vi "Create Paragraph Collection.vi"(8 "error in (no error)":errorcluster, 10 "Text":string, 11 "ooWriter in":refnum<class "ooWriter.lvclass">) -> (0 "error out":errorcluster, 2 "Paragraph Collection":refnum<k24>, 3 "ooWriter out":refnum<class "ooWriter.lvclass">)   [LabVIEW 2009, in "ooWriter.lvclass"]
uses:
  ooWriter.lvclass
  C:/Projets/LAVAG/OpenOfficeRGT/AODL/DLLs/AODL.dll
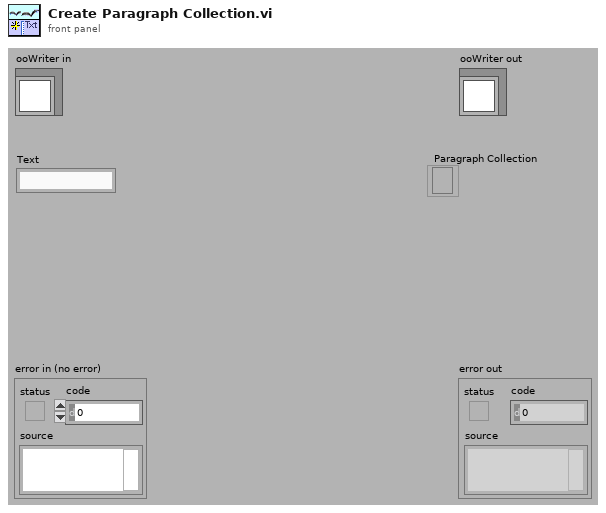
[diagram p1: front panel]
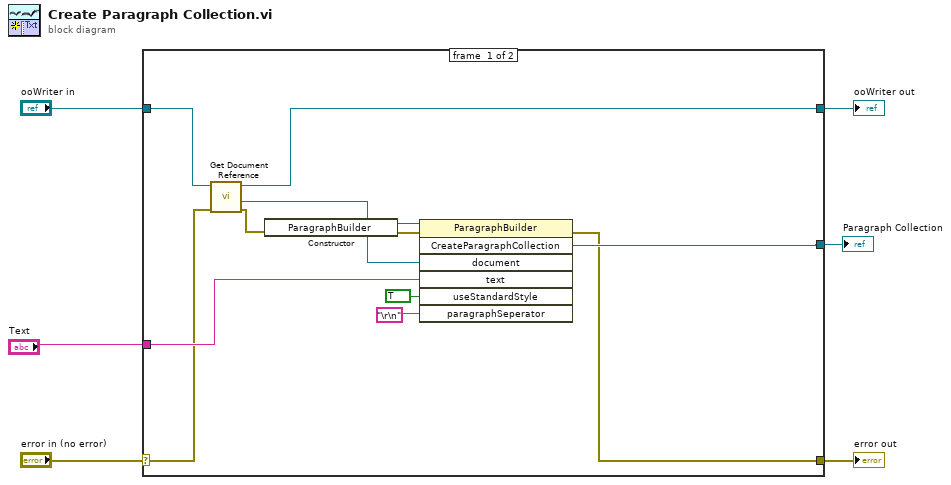
[diagram p0: block diagram]
diagram:
  n1 = case shown="No Error" "error in (no error)" {
    selector: "error in (no error)" -> [w8 w20]
    tunnel: [w7 w20] -> w5
    tunnel: [w10 w19] -> w3
    tunnel: "ooWriter in" -> [w11 w19]
    tunnel: "Text" -> [w16 _]
    tunnel: [w13 _] -> w1
    frame #0 {
      n2 = call-dynamic "Get Document Reference.vi"("error in (no error)"=w8, "ooDocument in"=w11) -> ("error out"=w9:errorcluster, "Document"=w12:refnum<k24>, "ooDocument out"=w10:refnum<class "ooWriter.lvclass">)  [unwired: 7 in]
      n3 = constructor class="ParagraphBuilder"(error in=w9) -> (reference out=w17:refnum<k24>, error out=w18:errorcluster)  [unwired: 2 in, 1 out]
      n4 = invoke class="ParagraphBuilder" method="CreateParagraphCollection"(reference=w17, error in=w18, "document"=w12, "text"=w16, "useStandardStyle"=TRUE, "paragraphSeperator"="\r\n") -> (error out=w7:errorcluster, "CreateParagraphCollection"=w13:refnum<k24>)  [unwired: 1 in, 5 out]
    }
    frame #1 {
    }
  }
  "error out" <- w5
  "ooWriter out" <- w3
  "Paragraph Collection" <- w1
